vi "Main - Password (1).vi"(8 "error in":errorcluster) -> (0 "error out":errorcluster, 3 "Pass?":bool)   [LabVIEW 2019]
uses:
  <userlib>/_OpenG.lib/md5/md5.llb/MD5 Message Digest (Hexadecimal String)__ogtk.vi
  <vilib>/httpClient/POSTBuffer.vi
  <vilib>/httpClient/LabVIEWHTTPClient.lvlib
panel:
  in  "Button":bool
  in  "Password":string
  # "Please Keyin Password"
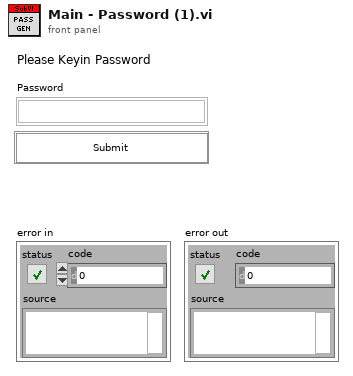
[diagram p1: front panel]
types:
  T1 = cluster{"action":string, "username":string, "password":string}
  T2 = cluster{"status":string, "data":cluster{"id":string, "username":string, "password":string, "delete":string}[]}
  T3 = typedef "eventvkey.ctl" = enum16{"ASCII", "Enter", "Return", "Shift", "Ctrl", "Alt", "Cmd", "Opt", "Caps", "NumLock", "Clear", "Break", "Up", "Down", "Left", "Right", "Insert", "Delete", "Home", "End", "PageUp", "PageDown", "Escape", "Help", "Pause", "ScrollLock", "F1", "F2", "F3", "F4", "F5", "F6", "F7", "F8", "F9", "F10", "F11", "F12", "F13", "F14", "F15", "F16", "F17", "F18", "F19", "F20", "F21", "F22", "F23", "F24", "Play", "VolumeUp", "VolumeDown", "Mute", "Two Byte Char"}
  T4 = typedef "LabVIEWHTTPClient.lvlib/ClientHandle.ctl" = refnum<k1>
  T5 = cluster{"id":string, "username":string, "password":string, "delete":string}[]
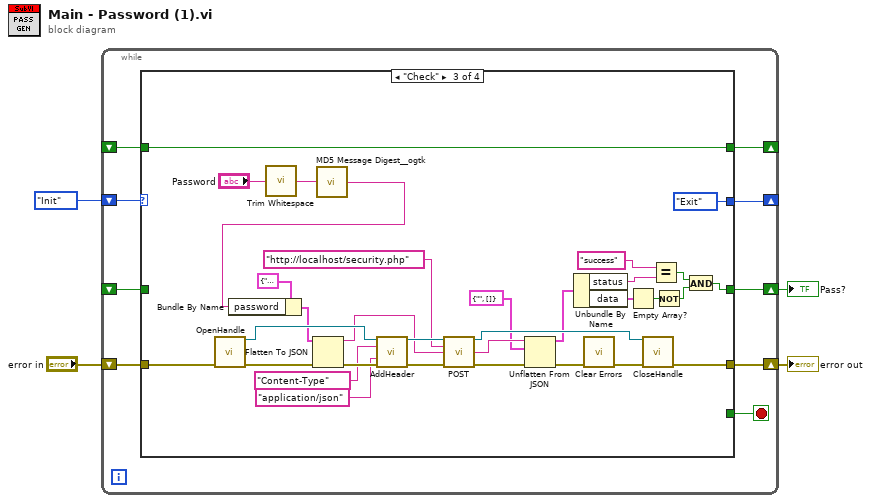
[diagram p0: block diagram]
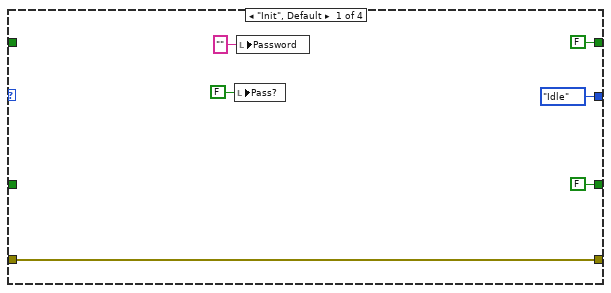
[diagram p2: hidden frame]
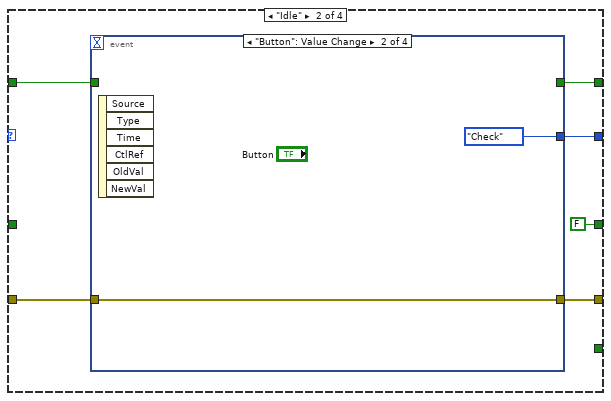
[diagram p3: hidden frame]
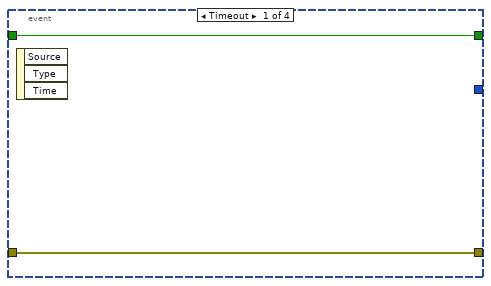
[diagram p4: hidden frame]
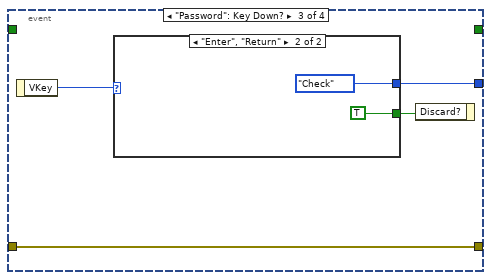
[diagram p5: hidden frame]
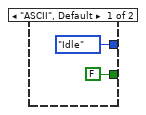
[diagram p6: hidden frame]
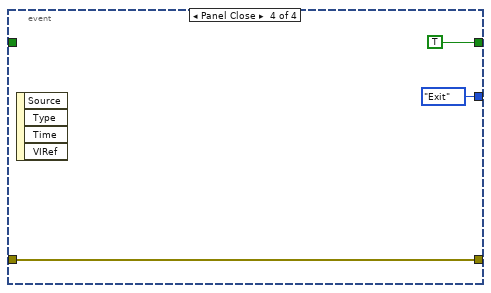
[diagram p7: hidden frame]
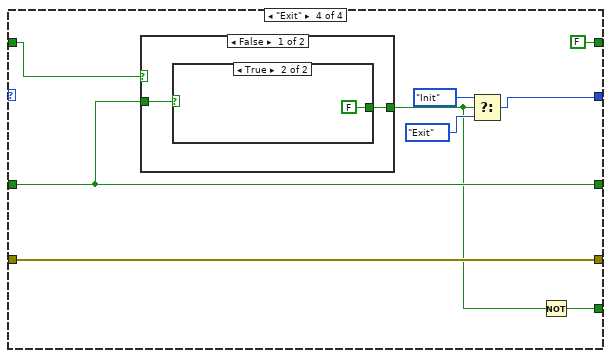
[diagram p8: hidden frame]
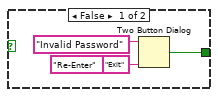
[diagram p9: hidden frame]
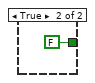
[diagram p10: hidden frame]
diagram:
  n1 = while {
    shift-right: [w12] -> _
    shift-left: enum16{"Init", "Idle", "Check", "Exit"}."Init" -> [w13]
    shift-right: [w11] -> w3
    shift-left: _ -> [w10]
    shift-right: [w8] -> w1
    shift-left: "error in" -> [w7]
    shift-right: [w6] -> _
    shift-left: _ -> [w5]
    stop <- w9 stop-if-true
    n2 = case shown="\"Check\"" w13 {
      tunnel: [enum16{"Init", "Idle", "Check", "Exit"}."Idle" w25 enum16{"Init", "Idle", "Check", "Exit"}."Exit" w76] -> w12
      tunnel: [FALSE FALSE w44 w80] -> w11
      tunnel: w10 -> [_ _ _ w80]
      tunnel: [_ _ _ w73] -> w9
      tunnel: [w15 w23 w45 w81] -> w8
      tunnel: w7 -> [w15 w22 w46 w81]
      tunnel: [FALSE w21 w71 FALSE] -> w6
      tunnel: w5 -> [_ w20 w71 w79]
      frame "Init", Default {
        n3 = local write "Pass?"(FALSE ("Pass?")) -> ()
        n4 = local write "Password"("" ("Password")) -> ()
      }
      frame "Idle" {
        n5 = event shown="[1] \"Button\": Value Change" {
          selector: _ -> [_ _ _ _]
          dyn-events: _ -> [_ _ _ _]
          timeout: _ -> [_ _ _ _]
          tunnel: [_ enum16{"Init", "Idle", "Check", "Exit"}."Check" w32 enum16{"Init", "Idle", "Check", "Exit"}."Exit"] -> w25
          tunnel: [w27 w28 w30 w40] -> w23
          tunnel: w22 -> [w27 w28 w30 w40]
          tunnel: [w26 _ _ TRUE] -> w21
          tunnel: w20 -> [w26 _ _ _]
          event Timeout {
            n6 = event-data() -> ()  [unwired: 1 in, 3 out]
          }
          event "Button": Value Change {
            n7 = event-data() -> ()  [unwired: 1 in, 6 out]
          }
          event "Password": Key Down? {
            n8 = event-data() -> ("VKey"=w33:T3)  [unwired: 1 in]
            n9 = case shown="\"Enter\", \"Return\"" w33 {
              tunnel: [enum16{"Init", "Idle", "Check", "Exit"}."Idle" enum16{"Init", "Idle", "Check", "Exit"}."Check"] -> w32
              tunnel: [FALSE TRUE] -> w31
              frame "ASCII", Default {
              }
              frame "Enter", "Return" {
              }
            }
            n10 = event-data("Discard?"=w31) -> ()  [unwired: 1 in, 1 out]
          }
          event Panel Close {
            n11 = event-data() -> ()  [unwired: 1 in, 4 out]
          }
        }
      }
      frame "Check" {
        n12 = call <vilib>:"OpenHandle.vi"("error in (no error)"=w46) -> ("client handle out"=w68:T4, "error out"=w69:errorcluster)  [unwired: 13 in]
        n13 = call <vilib>:"Trim Whitespace.vi"("string"="Password") -> ("trimmed string"=w42:string)  [unwired: 1 in]
        n14 = call-poly <userlib>:"MD5 Message Digest__ogtk.vi"("Message"=w42) -> ("MD5 Message Digest"=w43:string)
        n15 = Bundle By Name(cluster=T1 {"action"="read", "username"="geologic", "password"=""}, "password"=w43) -> (w61:T1)
        n16 = Flatten To JSON(anything=w61, error in (no error)=w69) -> (JSON string=w54:string, 11:w58:errorcluster)  [unwired: 1 in]
        n17 = call <vilib>:"AddHeader.vi"("client handle"=w68, "header"="Content-Type", "value"="application/json", "error in (no error)"=w58) -> ("client handle out"=w55:T4, "error out"=w56:errorcluster)  [unwired: 10 in]
        n18 = call-poly <vilib>:"POST.vi"("client handle"=w55, "url"="http://localhost/security.php", "buffer"=w54, "error in (no error)"=w56) -> ("client handle out"=w67:T4, "body"=w57:string, "error out"=w59:errorcluster)  [unwired: 8 in, 1 out]
        n19 = Unflatten From JSON(JSON string=w57, type and defaults=T2 {"status"="", "data"=[]}, error in (no error)=w59) -> (value=w53:T2, error out=w60:errorcluster)  [unwired: 4 in]
        n20 = Unbundle By Name(w53) -> ("status"=w63:string, "data"=w62:T5)
        n21 = call <vilib>:"Clear Errors.vi"("error in (no error)"=w60) -> ("error out"=w66:errorcluster)  [unwired: 5 in, 1 out]
        n22 = Empty Array?(array=w62) -> (empty?=w65:bool)
        n23 = call <vilib>:"CloseHandle.vi"("client handle"=w67, "error in (no error)"=w66) -> ("error out"=w45:errorcluster)  [unwired: 13 in]
        n24 = Equal?(x="success", y=w63) -> (x = y?=w64:bool)
        n25 = Not(x=w65) -> (.not. x?=w41:bool)
        n26 = And(x=w64, y=w41) -> (x .and. y?=w44:bool)
      }
      frame "Exit" {
        n27 = case shown="False" w79 {
          tunnel: w80 -> [w83 _]
          tunnel: [w82 FALSE ("T button?")] -> w74
          frame False {
            n28 = case shown="True" w83 {
              tunnel: [w85 FALSE ("T button?")] -> w82
              frame False {
                n29 = Two Button Dialog(message="Invalid Password", 1:"Exit" ("F button name (\"Cancel\")"), 2:"Re-Enter" ("T button name (\"OK\")")) -> (T button?=w85:bool)
              }
              frame True {
              }
            }
          }
          frame True {
          }
        }
        n30 = Select(t=enum16{"Init", "Idle", "Check", "Exit"}."Init", s=w74, f=enum16{"Init", "Idle", "Check", "Exit"}."Exit") -> (s? t:f=w76:enum16{"Init", "Idle", "Check", "Exit"})
        n31 = Not(x=w74) -> (.not. x?=w73:bool)
      }
    }
  }
  "Pass?" <- w3
  "error out" <- w1
